vi "labview python test vi.vi"() -> ()   [LabVIEW 2020]
panel:
  out "return value 2":dbl[](array[numeric])
  out "error out":errorcluster
  out "return value":u16[][](array[numeric])
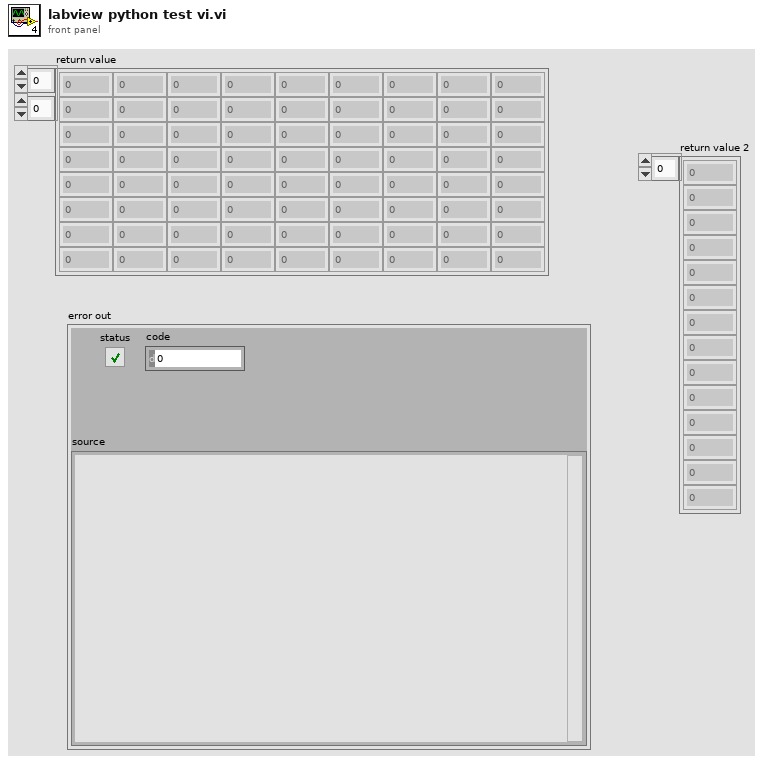
[diagram p1: front panel]
types:
  T1 = cluster{"Processed image":u16[][], "scalar results":dbl[]}
  T2 = typedef "IMAQ Image.ctl" = refnum<image>
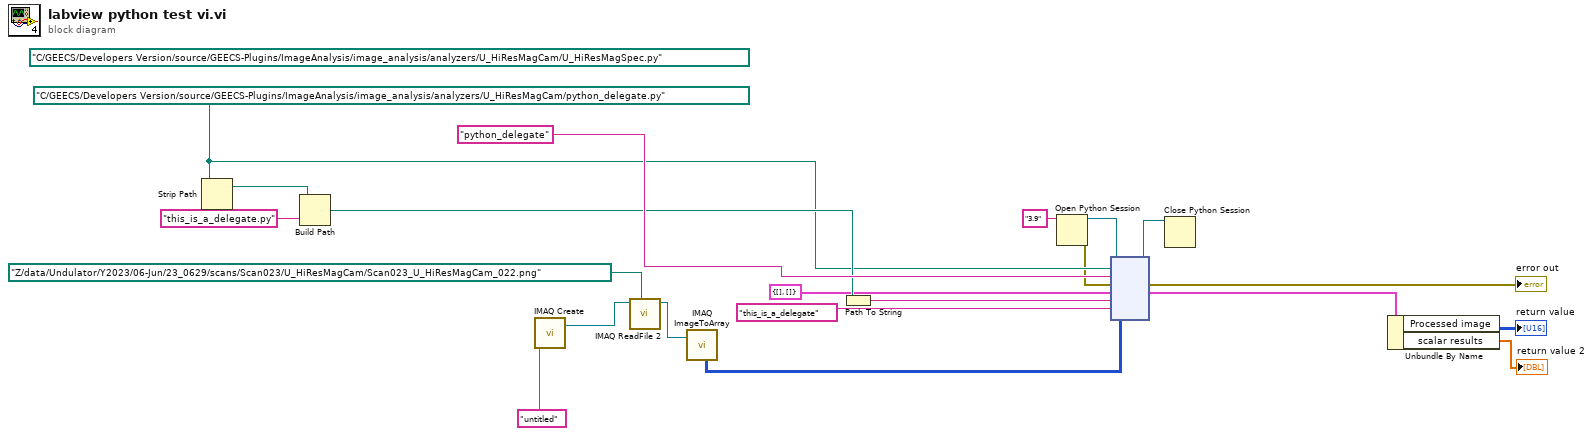
[diagram p0: block diagram]
diagram:
  (unwired) path "C:/GEECS/Developers Version/source/GEECS-Plugins/ImageAnalysis/image_analysis/analyzers/U_HiResMagCam/U_HiResMagSpec.py" ("PythonModulePath")
  w9 = path "C:/GEECS/Developers Version/source/GEECS-Plugins/ImageAnalysis/image_analysis/analyzers/U_HiResMagCam/python_delegate.py" ("PythonModulePath")
  n1 = Strip Path(path=w9) -> (stripped path=w11:path)  [unwired: 1 out]
  n2 = Build Path(base path=w11, name or relative path="this_is_a_delegate.py" ("PythonFunctionName")) -> (appended path=w13:path)
  n3 = call "IMAQ Create"("Image Name"="untitled") -> ("New Image"=w15:T2)  [unwired: 4 in, 1 out]
  n4 = call "IMAQ ReadFile 2"("File Path"=path "Z:/data/Undulator/Y2023/06-Jun/23_0629/scans/Scan023/U_HiResMagCam/Scan023_U_HiResMagCam_022.png", "Image"=w15) -> ("Image Out"=w14:T2)  [unwired: 5 in, 4 out]
  n5 = call "IMAQ ImageToArray"("Image"=w14) -> ("Image Pixels (U16)"=w6:u16[][])  [unwired: 3 in, 4 out]
  n6 = Path To String(path=w13) -> (string=w7:string)
  n7 = Open Python Session(python version="3.9" ("Python version")) -> (session out=w2:refnum<k35>, error out=w3:errorcluster)  [unwired: 2 in]
  n8 = node(w2, w9, "python_delegate" ("PythonFunctionName"), w3, T1 {"Processed image"=[], "scalar results"=[]}, w7, "this_is_a_delegate" ("PythonFunctionName"), w6) -> (w1:refnum<k35>, →"error out":errorcluster, w5:T1)  [unwired: 3 in, 2 out]
  n9 = Close Python Session(session in=w1) -> ()  [unwired: 1 in, 1 out]
  n10 = Unbundle By Name(w5) -> ("Processed image"=→"return value":u16[][], "scalar results"=→"return value 2":dbl[])
